vi "Func - FuncVI Refnums (Open Clone).vi"(6 "cmd (get)":enum16{"get", "close inst", "close all"}(ring), 7 "Func Info in":T1, 8 "error in":errorcluster, 11 "Instance ID":u64 format="%.0x") -> (0 "error out":errorcluster, 2 "FuncVI2 RefNum":refnum<vi>, 3 "FuncVI RefNum":refnum<vi>)   [LabVIEW 2021]
doc: "::: CalcExpress Toolkit :::\nCopyright (c) 2000-2026 Konstantin Shifershteyn. All rights reserved."
panel:
  in  "FuncVI2 RefNum Template":refnum<vi>
  in  "FuncVI RefNum Template":refnum<vi>
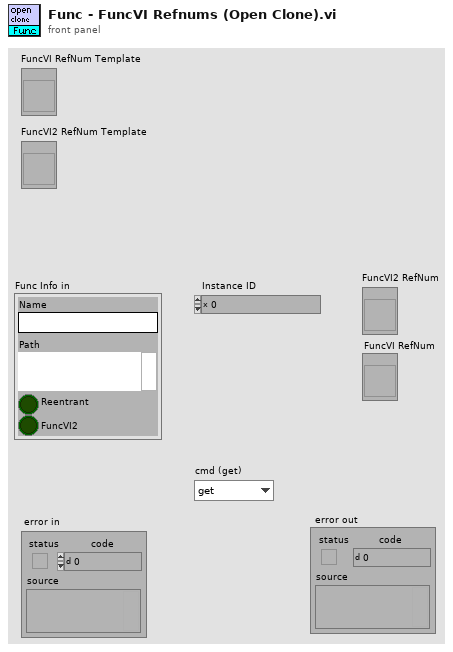
[diagram p1: front panel]
types:
  T1 = cluster{"Name":string, "Path":path, "Reentrant":bool, "FuncVI2":bool}
  T2 = cluster{"FuncVI RefNum Template":refnum<vi>, "FuncVI2 RefNum Template":refnum<vi>}
  T3 = cluster{"FuncVI RefNum Template":refnum<vi>, "FuncVI2 RefNum Template":refnum<vi>}[]
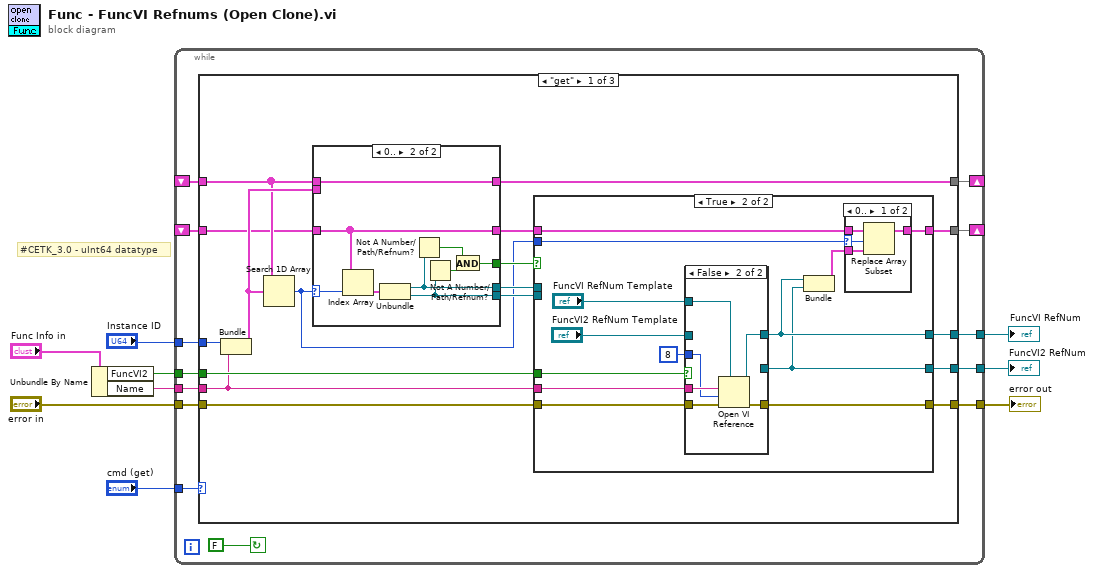
[diagram p0: block diagram]
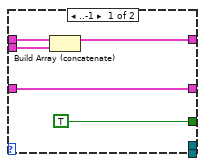
[diagram p2: hidden frame]
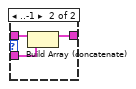
[diagram p4: hidden frame]
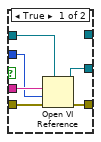
[diagram p5: hidden frame]
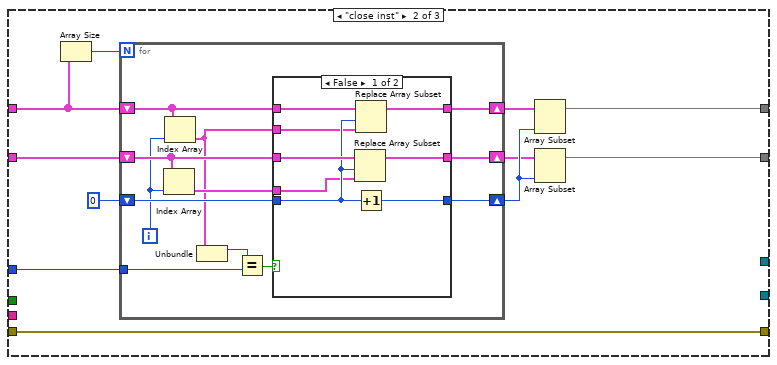
[diagram p6: hidden frame]
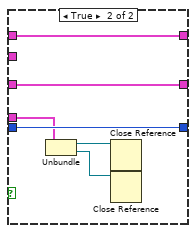
[diagram p7: hidden frame]
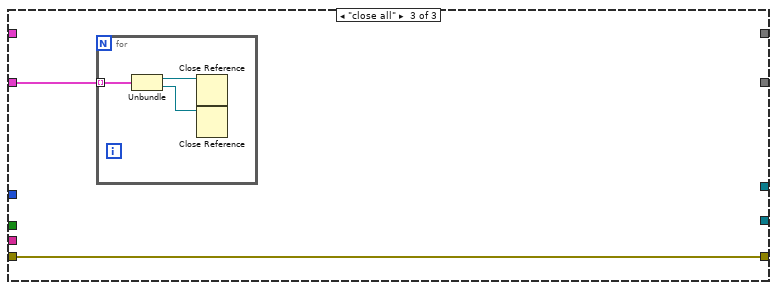
[diagram p8: hidden frame]
diagram:
  # "#CETK_3.0 - uInt64 datatype"
  n1 = Unbundle By Name("Func Info in") -> ("FuncVI2"=w3:bool, "Name"=w4:string)
  n2 = while {
    tunnel: [w22] -> w9
    tunnel: [w21] -> w8
    tunnel: [w20] -> w7
    tunnel: "error in" -> [w19]
    tunnel: w4 -> [w18]
    tunnel: w3 -> [w17]
    tunnel: "cmd (get)" -> [w15]
    shift-right: [w13] -> _
    shift-left: _ -> [w14]
    tunnel: "Instance ID" -> [w12]
    shift-right: [w10] -> _
    shift-left: _ -> [w11]
    stop <- FALSE continue-if-true
    n3 = case shown="\"get\"" w15 {
      tunnel: [w36 _ _] -> w22
      tunnel: [w39 w100 w128] -> w21
      tunnel: [w35 _ _] -> w20
      tunnel: w19 -> [w38 w100 w128]
      tunnel: w18 -> [w32 _ _]
      tunnel: w17 -> [w37 _ _]
      tunnel: w14 -> [w28 w99 w127]
      tunnel: [w34 w90 _] -> w13
      tunnel: w12 -> [w33 w96 _]
      tunnel: w11 -> [w29 w98 _]
      tunnel: [w31 w91 _] -> w10
      frame "get" {
        n4 = Bundle("Instance ID"=w33, "Name"=w32) -> (w30:cluster{"Instance ID":u64, "Name":string})  [unwired: 1 in]
        n5 = Search 1D Array(1D array=w29, element=w30) -> (index of element=w23:i32)  [unwired: 1 in]
        n6 = case shown="0.." w23 {
          selector: w23 -> [_ w51]
          tunnel: [w44 w53] -> w31
          tunnel: w30 -> [w43 _]
          tunnel: w29 -> [w42 w53]
          tunnel: w28 -> [w41 w50]
          tunnel: [w41 w50] -> w27
          tunnel: [TRUE w47] -> w26
          tunnel: [_ w46] -> w25
          tunnel: [_ w45] -> w24
          frame ..-1 {
            n7 = Build Array (concatenate)(w42, w43) -> (w44:cluster{"Instance ID":u64, "Name":string}[])
          }
          frame 0.. {
            n8 = Index Array(array=w50, index=w51) -> (element=w52:T2)
            n9 = Unbundle(w52) -> ("FuncVI RefNum Template"=w46:refnum<vi>, "FuncVI2 RefNum Template"=w45:refnum<vi>)
            n10 = Not A Number/Path/Refnum?(number/path/refnum=w46) -> (NaN/Path/Refnum?=w49:bool)
            n11 = Not A Number/Path/Refnum?(number/path/refnum=w45) -> (NaN/Path/Refnum?=w48:bool)
            n12 = And(x=w49, y=w48) -> (x .and. y?=w47:bool)
          }
        }
        n13 = case shown="True" w26 {
          tunnel: [w55 w70] -> w39
          tunnel: w38 -> [w55 w69]
          tunnel: w37 -> [_ w68]
          tunnel: [w57 w67] -> w36
          tunnel: [w56 w66] -> w35
          tunnel: w27 -> [w54 w65]
          tunnel: [w54 w64] -> w34
          tunnel: w32 -> [_ w63]
          tunnel: w23 -> [_ w58]
          tunnel: w25 -> [w57 _]
          tunnel: w24 -> [w56 _]
          frame False {
          }
          frame True {
            n14 = case shown="False" w68 {
              tunnel: w69 -> [w83 w89]
              tunnel: [w81 w87] -> w70
              tunnel: w63 -> [w82 w88]
              tunnel: [w78 _] -> w66
              tunnel: "FuncVI2 RefNum Template" -> [w80 _]
              tunnel: 8 ("options") -> [w79 w86]
              tunnel: [_ w85] -> w67
              tunnel: "FuncVI RefNum Template" -> [_ w84]
              frame True {
                n15 = Open VI Reference(type specifier VI Refnum (for type only)=w80, vi path=w82, options=w79, error in (no error)=w83) -> (vi reference=w78:refnum<vi>, error out=w81:errorcluster)  [unwired: 2 in]
              }
              frame False {
                n16 = Open VI Reference(type specifier VI Refnum (for type only)=w84, vi path=w88, options=w86, error in (no error)=w89) -> (vi reference=w85:refnum<vi>, error out=w87:errorcluster)  [unwired: 2 in]
              }
            }
            n17 = Bundle("FuncVI RefNum Template"=w67, "FuncVI2 RefNum Template"=w66) -> (w59:T2)  [unwired: 1 in]
            n18 = case shown="0.." w58 {
              selector: w58 -> [w71 _]
              tunnel: w65 -> [w74 w77]
              tunnel: [w73 w76] -> w64
              tunnel: w59 -> [w72 w75]
              frame 0.. {
                n19 = Replace Array Subset(array=w74, new element=w72, index=w71) -> (w73:T3)
              }
              frame ..-1 {
                n20 = Build Array (concatenate)(w77, w75) -> (w76:T3)
              }
            }
          }
        }
      }
      frame "close inst" {
        n21 = Array Size(array=w98) -> (size(s)=w97:i32)
        n22 = for {
          N: w97 -> [_]
          shift-right: [w108] -> w92
          shift-left: w98 -> [w109]
          shift-right: [w107] -> w93
          shift-left: w99 -> [w104]
          tunnel: w96 -> [w112]
          shift-right: [w105] -> w94
          shift-left: 0 -> [w106]
          i -> [w103]
          n23 = Index Array(array=w104, index=w103) -> (element=w102:T2)
          n24 = Index Array(array=w109, index=w103) -> (element=w101:cluster{"Instance ID":u64, "Name":string})
          n25 = Unbundle(w101) -> ("Instance ID"=w111:u64)  [unwired: 1 out]
          n26 = Equal?(x=w111, y=w112) -> (x = y?=w110:bool)
          n27 = case shown="False" w110 {
            tunnel: w109 -> [w119 w126]
            tunnel: [w118 w126] -> w108
            tunnel: w104 -> [w120 w124]
            tunnel: [w117 w124] -> w107
            tunnel: w106 -> [w115 w125]
            tunnel: [w116 w125] -> w105
            tunnel: w102 -> [w114 w121]
            tunnel: w101 -> [w113 _]
            frame False {
              n28 = Replace Array Subset(array=w120, new element=w114, index=w115) -> (w117:T3)
              n29 = Replace Array Subset(array=w119, new element=w113, index=w115) -> (w118:cluster{"Instance ID":u64, "Name":string}[])
              n30 = Increment(x=w115) -> (x+1=w116:i32)
            }
            frame True {
              n31 = Unbundle(w121) -> ("FuncVI RefNum Template"=w123:refnum<vi>, "FuncVI2 RefNum Template"=w122:refnum<vi>)
              n32 = Close Reference(reference=w123) -> ()  [unwired: 1 in, 1 out]
              n33 = Close Reference(reference=w122) -> ()  [unwired: 1 in, 1 out]
            }
          }
        }
        n34 = Array Subset(array=w92, length=w94) -> (w91:cluster{"Instance ID":u64, "Name":string}[])  [unwired: 1 in]
        n35 = Array Subset(array=w93, length=w94) -> (w90:T3)  [unwired: 1 in]
      }
      frame "close all" {
        n36 = for {
          tunnel: w127 -> [w129] mode=indexing
          n37 = Unbundle(w129) -> ("FuncVI RefNum Template"=w131:refnum<vi>, "FuncVI2 RefNum Template"=w130:refnum<vi>)
          n38 = Close Reference(reference=w131) -> ()  [unwired: 1 in, 1 out]
          n39 = Close Reference(reference=w130) -> ()  [unwired: 1 in, 1 out]
        }
      }
    }
  }
  "error out" <- w8
  "FuncVI RefNum" <- w9
  "FuncVI2 RefNum" <- w7
